vi "module id update test.vi"() -> (0 "error out":errorcluster, 2 "Pass":bool)   [LabVIEW 2014, in "execution interface tests.lvlib"]
uses:
  execution interface tests.lvlib
  Engine Configuration/engine configuration.lvclass
  <vilib>/NI/Tag Bus/tag/Data Type.ctl
  <vilib>/NI/Tag Bus Module Framework/channel/channel classification.ctl
  <vilib>/NI/Tag Bus/tag/tag descriptor.lvclass
  <vilib>/NI/Tag Bus Module Framework/channel/TBM channel.lvclass
panel:
  out "engine configuration out":refnum<class "engine configuration.lvclass">
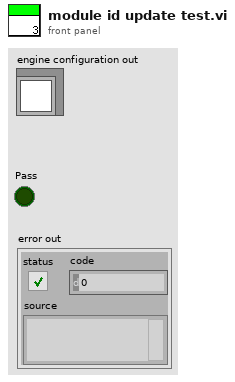
[diagram p1: front panel]
types:
  T1 = typedef "TBM channel.lvclass/channel classification.ctl" = enum16{"input data", "output data", "processing parameter", "processing result"}
  T2 = typedef "tag bus.lvlib/tag descriptor.lvclass/Data Type.ctl" = enum16{"Double", "Single", "I64", "I32", "I16", "I8", "U64", "U32", "U16", "U8", "Boolean", "String", "Array of Double", "Array of Single", "Array of I64", "Array of I32", "Array of I16", "Array of I8", "Array of U64", "Array of U32", "Array of U16", "Array of U8", "Array of Boolean", "Array of String"}
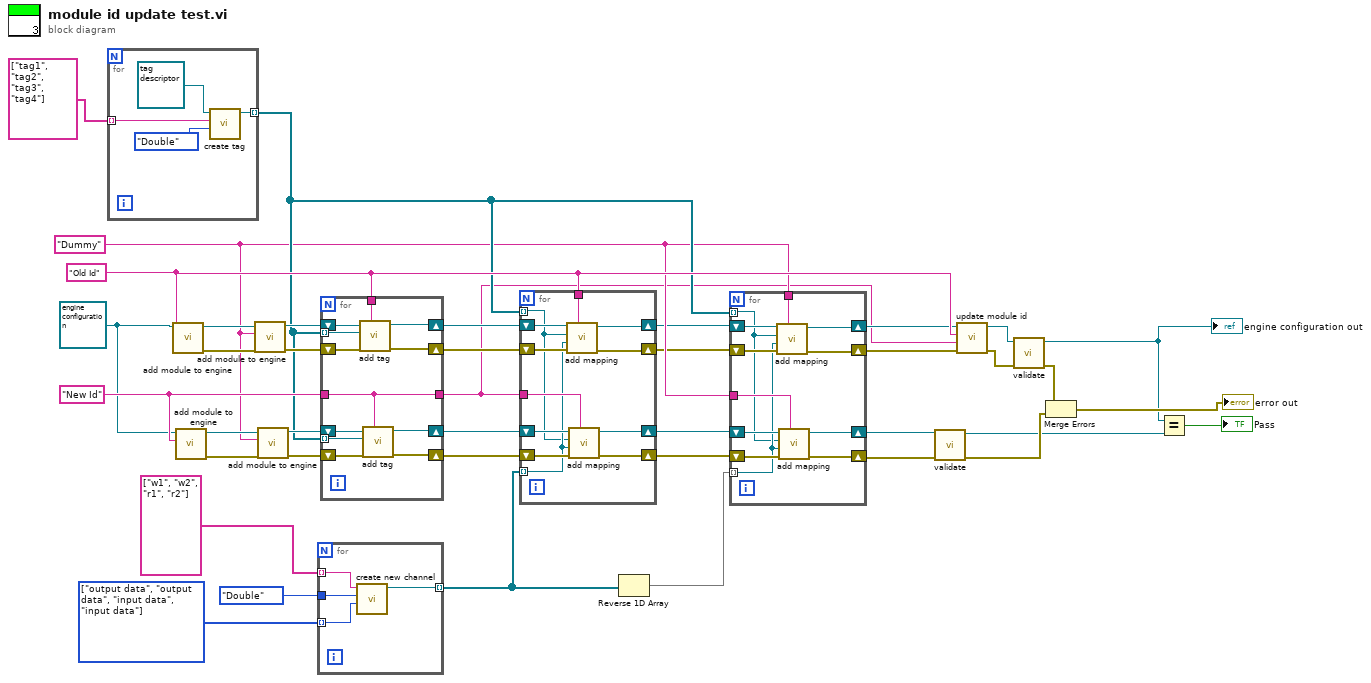
[diagram p0: block diagram]
diagram:
  w27 = T1[] [enum."output data", enum."output data", enum."input data", enum."input data"] items=["input data", "output data", "processing parameter", "processing result"]
  w32 = "New Id" ("New Id")
  w23 = "Old Id" ("Old Id")
  w17 = "Dummy" ("module ID")
  w31 = refnum<class "engine configuration.lvclass"> refnum ("engine configuration")
  n1 = for {
    tunnel: [w42] -> w18 mode=indexing
    tunnel: string[] ["tag1", "tag2", "tag3", "tag4"] -> [w41] mode=indexing
    n2 = call-dynamic "create tag.vi"("data type"=Data_Type."Double", "name"=w41, "tag descriptor in"=refnum<class "tag descriptor.lvclass"> refnum) -> ("tag descriptor out"=w42:refnum<class "tag descriptor.lvclass">)  [unwired: 7 in, 1 out]
  }
  n3 = call-dynamic "add module to engine.vi"("module ID"=w23, "engine configuration in"=w31) -> ("error out"=w38:errorcluster, "engine configuration out"=w40:refnum<class "engine configuration.lvclass">)  [unwired: 8 in]
  n4 = call-dynamic "add module to engine.vi"("module ID"=w32, "engine configuration in"=w31) -> ("error out"=w35:errorcluster, "engine configuration out"=w33:refnum<class "engine configuration.lvclass">)  [unwired: 8 in]
  n5 = call-dynamic "add module to engine.vi"("error in"=w38, "module ID"=w17, "engine configuration in"=w40) -> ("error out"=w37:errorcluster, "engine configuration out"=w39:refnum<class "engine configuration.lvclass">)  [unwired: 7 in]
  n6 = call-dynamic "add module to engine.vi"("error in"=w35, "module ID"=w17, "engine configuration in"=w33) -> ("error out"=w36:errorcluster, "engine configuration out"=w34:refnum<class "engine configuration.lvclass">)  [unwired: 7 in]
  n7 = for {
    tunnel: string[] ["w1", "w2", "r1", "r2"] -> [w46] mode=indexing
    tunnel: w27 -> [w47] mode=indexing
    tunnel: Data_Type."Double" ("data type") -> [w48]
    tunnel: [w45] -> w20 mode=indexing
    n8 = call <vilib>:"create new channel.vi"("channel classification"=w47, "data type"=w48, "channel name"=w46) -> ("channel"=w45:refnum<class "TBM channel.lvclass">)  [unwired: 8 in]
  }
  n9 = for {
    tunnel: w32 -> [w50]
    shift-right: [w53] -> w25
    shift-left: w39 -> [w60]
    shift-right: [w54] -> w22
    shift-left: w37 -> [w59]
    shift-right: [w55] -> w24
    shift-left: w34 -> [w57]
    shift-right: [w56] -> w21
    shift-left: w36 -> [w58]
    tunnel: w18 -> [w52] mode=indexing
    tunnel: w18 -> [w51] mode=indexing
    tunnel: w23 -> [w49]
    tunnel: [w50] -> w9
    n10 = call-dynamic "add tag.vi"("owner ID"=w49, "error in"=w59, "tag descriptor"=w52, "engine configuration in"=w60) -> ("error out"=w54:errorcluster, "engine configuration out"=w53:refnum<class "engine configuration.lvclass">)  [unwired: 6 in]
    n11 = call-dynamic "add tag.vi"("owner ID"=w50, "error in"=w58, "tag descriptor"=w51, "engine configuration in"=w57) -> ("error out"=w56:errorcluster, "engine configuration out"=w55:refnum<class "engine configuration.lvclass">)  [unwired: 6 in]
  }
  n12 = for {
    shift-right: [w69] -> w16
    shift-left: w25 -> [w72]
    shift-right: [w70] -> w14
    shift-left: w24 -> [w71]
    tunnel: w23 -> [w68]
    shift-right: [w64] -> w15
    shift-left: w22 -> [w67]
    shift-right: [w65] -> w13
    shift-left: w21 -> [w66]
    tunnel: w9 -> [w63]
    tunnel: w20 -> [w62] mode=indexing
    tunnel: w18 -> [w61] mode=indexing
    n13 = call-dynamic "add mapping.vi"("owner ID"=w68, "error in"=w67, "channel"=w62, "tag descriptor"=w61, "engine configuration"=w72) -> ("error out"=w64:errorcluster, "engine configuration out"=w69:refnum<class "engine configuration.lvclass">)  [unwired: 5 in]
    n14 = call-dynamic "add mapping.vi"("owner ID"=w63, "error in"=w66, "channel"=w62, "tag descriptor"=w61, "engine configuration"=w71) -> ("error out"=w65:errorcluster, "engine configuration out"=w70:refnum<class "engine configuration.lvclass">)  [unwired: 5 in]
  }
  n15 = Reverse 1D Array(array=w20) -> (reversed array=w19:refnum<class "TBM channel.lvclass">[])
  n16 = for {
    shift-right: [w81] -> w10
    shift-left: w16 -> [w84]
    shift-right: [w82] -> w4
    shift-left: w14 -> [w83]
    tunnel: w17 -> [w80]
    shift-right: [w76] -> w12
    shift-left: w15 -> [w79]
    shift-right: [w77] -> w3
    shift-left: w13 -> [w78]
    tunnel: w17 -> [w75]
    tunnel: w19 -> [w74] mode=indexing
    tunnel: w18 -> [w73] mode=indexing
    n17 = call-dynamic "add mapping.vi"("owner ID"=w80, "error in"=w79, "channel"=w74, "tag descriptor"=w73, "engine configuration"=w84) -> ("error out"=w76:errorcluster, "engine configuration out"=w81:refnum<class "engine configuration.lvclass">)  [unwired: 5 in]
    n18 = call-dynamic "add mapping.vi"("owner ID"=w75, "error in"=w78, "channel"=w74, "tag descriptor"=w73, "engine configuration"=w83) -> ("error out"=w77:errorcluster, "engine configuration out"=w82:refnum<class "engine configuration.lvclass">)  [unwired: 5 in]
  }
  n19 = call-dynamic "validate.vi"("error in"=w3, "configuration in"=w4) -> ("error out"=w2:errorcluster, "configuration out"=w1:refnum<class "engine configuration.lvclass">)  [unwired: 8 in]
  n20 = call-dynamic "update module id.vi"("error in (no error)"=w12, "New Id"=w9, "Old Id"=w23, "engine configuration in"=w10) -> ("error out"=w8:errorcluster, "engine configuration out"=w6:refnum<class "engine configuration.lvclass">)  [unwired: 6 in]
  n21 = call-dynamic "validate.vi"("error in"=w8, "configuration in"=w6) -> ("error out"=w7:errorcluster, "configuration out"=w5:refnum<class "engine configuration.lvclass">)  [unwired: 8 in]
  "engine configuration out" <- w5
  n22 = Merge Errors(w7, w2) -> (→"error out":errorcluster)
  n23 = Equal?(x=w5, y=w1) -> (x = y?=→"Pass":bool)
